vi "Concurrency.vi"() -> ()   [LabVIEW 2026]
panel:
  out "Numeric":i32
  out "Count Complete":bool
  out "Read Complete":bool
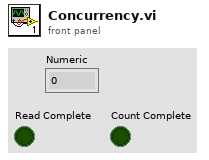
[diagram p1: front panel]
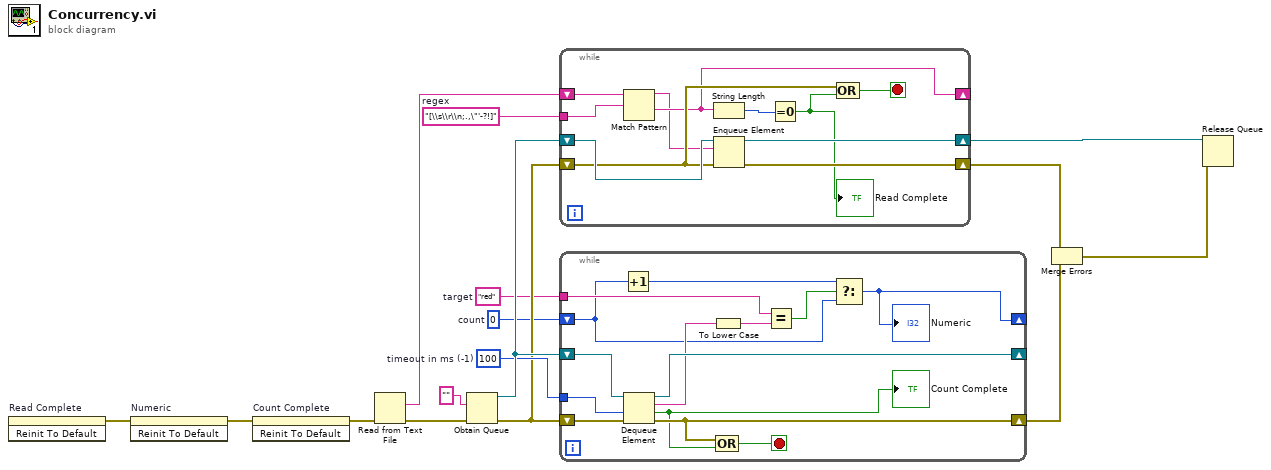
[diagram p0: block diagram]
diagram:
  w5 = "[\\s\\r\\n;.,\"'-?!]"  # regex
  w7 = 0  # count
  w10 = 100  # timeout in ms (-1)
  w8 = "red"  # target
  n1 = invoke on="Read Complete" class="Bool (strict)" method="Reinit To Default"() -> (error out=w15:errorcluster)  [unwired: 3 in, 2 out]
  n2 = invoke on="Numeric" class="DigNum (strict)" method="Reinit To Default"(error in=w15) -> (error out=w14:errorcluster)  [unwired: 2 in, 2 out]
  n3 = invoke on="Count Complete" class="Bool (strict)" method="Reinit To Default"(error in=w14) -> (error out=w13:errorcluster)  [unwired: 2 in, 2 out]
  n4 = Read from Text File(error in=w13) -> (text=w6:string, error out=w16:errorcluster)  [unwired: 3 in, 2 out]
  n5 = Obtain Queue(element data type="", error in (no error)=w16) -> (queue out=w11:refnum<queue>, error out=w9:errorcluster)  [unwired: 3 in, 1 out]
  n6 = while {
    shift-right: [w27] -> w3
    shift-left: w9 -> [w23]
    shift-right: [w25] -> w12
    shift-left: w11 -> [w26]
    shift-right: [w21] -> _
    shift-left: w6 -> [w22]
    tunnel: w5 -> [w18]
    stop <- w24 stop-if-true
    n7 = Match Pattern(string=w22, regular expression=w18) -> (before substring=w19:string, after substring=w21:string)  [unwired: 1 in, 2 out]
    n8 = String Length(string=w21) -> (length=w20:i32)
    n9 = Enqueue Element(queue=w26, element=w19, error in (no error)=w23) -> (queue out=w25:refnum<queue>, error out=w27:errorcluster)  [unwired: 1 in, 1 out]
    n10 = Equal To 0?(x=w20) -> (x = 0?=w17:bool)
    "Read Complete" <- w17
    n11 = Compound Arithmetic op=OR(w23, w17) -> (w24:bool)
  }
  n12 = while {
    shift-right: [w38] -> _
    shift-left: w11 -> [w41]
    tunnel: w10 -> [w40]
    shift-right: [w36] -> w2
    shift-left: w9 -> [w39]
    tunnel: w8 -> [w32]
    shift-right: [w28] -> _
    shift-left: w7 -> [w29]
    stop <- w37 stop-if-true
    n13 = Increment(x=w29) -> (x+1=w30:i32)
    n14 = Dequeue Element(queue=w41, timeout in ms (-1)=w40, error in (no error)=w39) -> (queue out=w38:refnum<queue>, element=w34:string, timed out?=w35:bool, error out=w36:errorcluster)
    "Count Complete" <- w35
    n15 = To Lower Case(string=w34) -> (all lower case string=w33:string)
    n16 = Compound Arithmetic op=OR(w36, w35) -> (w37:bool)
    n17 = Equal?(x=w32, y=w33) -> (x = y?=w31:bool)
    n18 = Select(t=w30, s=w31, f=w29) -> (s? t:f=w28:i32)
    "Numeric" <- w28
  }
  n19 = Merge Errors(w3, w2) -> (w1:errorcluster)
  n20 = Release Queue(queue=w12, error in (no error)=w1) -> ()  [unwired: 1 in, 3 out]
